vi "To and  From CSV.vi"() -> (0 "error out":errorcluster, 3 "Pass":bool)   [LabVIEW 2015, in "DAQmx Module Tests.lvlib"]
uses:
  DAQmx Module Tests.lvlib
  <vilib>/NI/Module Execution Interface/Engine Configuration/engine configuration.lvclass
  editor node/DAQmx Module editor node.lvclass
  <vilib>/NI/Configuration Framework/serializable configuration/NISE_CEF_serializable configuration.lvclass/NISE_CEF_serializable configuration.ctl
  module/configuration/Daqmx Module configuration.lvclass/Daqmx Module configuration.ctl
  <vilib>/Utility/LVClass/Get LV Class Name.vi
  <vilib>/NI/Configuration Framework/error generator/NISE_error generator.vi
  <vilib>/NI/Tag Bus Module Framework/channel/TBM channel.lvclass
  module/configuration/Daqmx Module configuration.lvclass
  <vilib>/NI/Configuration Framework/serializable configuration/NISE_CEF_serializable configuration.lvclass
panel:
  out "Object":bool
  out "Lines":bool
  out "Write Channels":bool
  out "Read Channels":bool
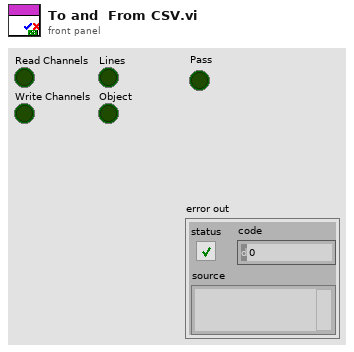
[diagram p1: front panel]
types:
  T1 = typedef "DAQmx Module Configuration.lvclass/Line.ctl" = cluster{"Channel Array":refnum<class "TBM channel.lvclass">[], "Physical Channel":string, "Measurement Type":T2, "Parameters":T3}
  T2 = typedef "DAQmx Module Configuration.lvclass/Measurement Type.ctl" = enum16{"Digital Input", "Digital Output", "Voltage Input", "Voltage Output", "Current Input", "Current Output", "RTD", "Thermocouple", "Strain", "PWM"}
  T3 = typedef "DAQmx Module Configuration.lvclass/Parameters.ctl" = cluster{"Digital Config":cluster{"Invert Lines?":bool}, "Voltage Config":cluster{"Maximum Value (V)":dbl, "Minimum Value (V)":dbl, "in terminal configuration (V)":i32, "out terminal configuration (V)":i32}, "Current Config":cluster{"Maximum Value (A)":dbl, "Minimum Value (A)":dbl, "shunt resistor location":i32, "input terminal configuration (C)":i32, "external shunt resistor value":dbl}, "RTD Config":cluster{"Maximum Value (°C)":dbl, "Minimum Value (°C)":dbl, "resistance configuration":i32, "r0":dbl, "current excitation value":dbl, "rtd type":i32, "current excitation source":i32}, "Thermocouple Config":cluster{"Minimum Value (C)":dbl, "Maximum Value (C)":dbl, "thermocouple type":i32, "cjc source":i32, "cjc value":dbl}, "Strain Config":cluster{"Maximum Value":dbl, "Minimum Value":dbl, "bridge information":cluster{"strain configuration":i32, "lead wire resistance":dbl, "initial bridge voltage":dbl, "voltage excitation source":i32, "voltage excitation value":dbl}, "strain gage information":cluster{"gage factor":dbl, "nominal gage resistance":dbl, "poisson ratio":dbl}}, "PWM Config":cluster{"Idle State":bool}}
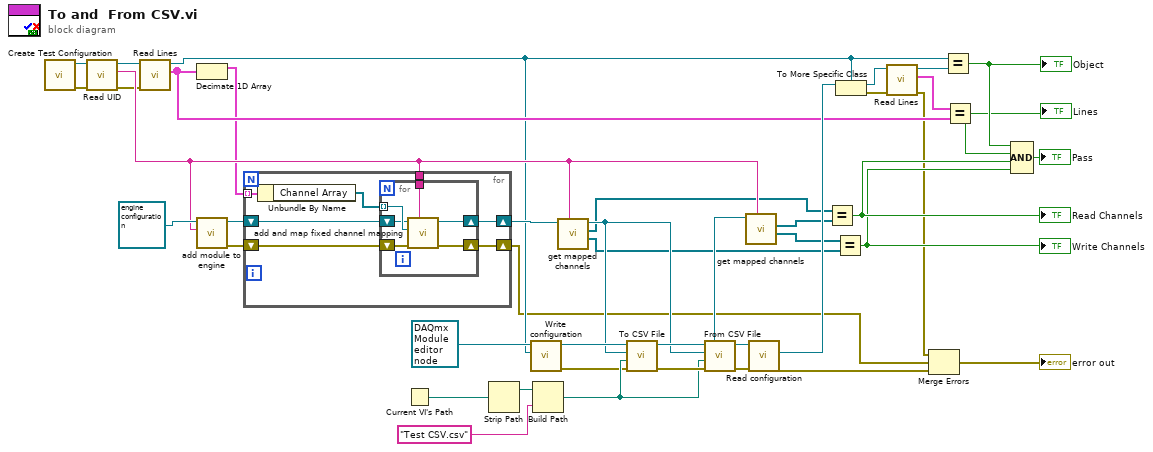
[diagram p0: block diagram]
diagram:
  n1 = call "Create Test Configuration.vi"() -> ("error out"=w17:errorcluster, "Module Configuration"=w27:refnum<class "Daqmx Module configuration.lvclass">)  [unwired: 7 in, 3 out]
  n2 = call <vilib>:"Read UID.vi"("error in"=w17, "configuration in"=w27) -> ("error out"=w13:errorcluster, "instance id"=w23:string, "configuration out"=w16:refnum<class "Daqmx Module configuration.lvclass">)  [unwired: 7 in]
  n3 = call "Read Lines.vi"("error in (no error)"=w13, "Daqmx Module configuration in"=w16) -> ("Lines"=w30:T1[], "Daqmx Module configuration out"=w15:refnum<class "Daqmx Module configuration.lvclass">)  [unwired: 7 in, 1 out]
  n4 = Decimate 1D Array(w30) -> (w18:T1[])  [unwired: 1 out]
  n5 = call-dynamic "add module to engine.vi"("module ID"=w23, "engine configuration in"=refnum<class "engine configuration.lvclass"> refnum ("engine configuration")) -> ("error out"=w12:errorcluster, "engine configuration out"=w28:refnum<class "engine configuration.lvclass">)  [unwired: 8 in]
  n6 = for {
    tunnel: w18 -> [w50] mode=indexing
    shift-right: [w48] -> w26
    shift-left: w28 -> [w47]
    tunnel: w23 -> [w46]
    shift-right: [w44] -> w9
    shift-left: w12 -> [w45]
    n7 = Unbundle By Name(w50) -> ("Channel Array"=w49:refnum<class "TBM channel.lvclass">[])
    n8 = for {
      tunnel: w49 -> [w56] mode=indexing
      tunnel: w46 -> [w53]
      shift-right: [w55] -> w48
      shift-left: w47 -> [w54]
      shift-right: [w51] -> w44
      shift-left: w45 -> [w52]
      n9 = call <vilib>:"add and map fixed channel mapping.vi"("module instance"=w53, "error in"=w52, "fixed channel"=w56, "engine configuration in"=w54) -> ("error out"=w51:errorcluster, "engine configuration out"=w55:refnum<class "engine configuration.lvclass">)  [unwired: 6 in]
    }
  }
  n10 = Current VI's Path() -> (path=w20:path)
  n11 = Strip Path(path=w20) -> (stripped path=w19:path)  [unwired: 1 out]
  n12 = call-dynamic "Write configuration.vi"("configuration"=w15, "Daqmx Module editor node in"=refnum<class "DAQmx Module editor node.lvclass"> refnum ("Daqmx Module editor node")) -> ("error out"=w5:errorcluster, "Daqmx Module editor node out"=w35:refnum<class "DAQmx Module editor node.lvclass">)  [unwired: 8 in]
  n13 = Build Path(base path=w19, name or relative path="Test CSV.csv") -> (appended path=w21:path)
  n14 = call-dynamic "get mapped channels.vi"("owner"=w23, "engine configuration in"=w26) -> ("write channels"=w4:refnum<class "TBM channel.lvclass">[], "read channels"=w3:refnum<class "TBM channel.lvclass">[], "engine configuration out"=w25:refnum<class "engine configuration.lvclass">)  [unwired: 5 in, 2 out]
  n15 = call-dynamic "To CSV File.vi"("error in (no error)"=w5, "Path"=w21, "engine configuration"=w25, "DAQmx Module Editor Node in"=w35) -> ("error out"=w38:errorcluster, "DAQmx Module Editor Node out"=w37:refnum<class "DAQmx Module editor node.lvclass">)  [unwired: 6 in]
  n16 = call-dynamic "From CSV File.vi"("error in (no error)"=w38, "Path"=w21, "engine configuration"=w25, "DAQmx Module Editor Node in"=w37) -> ("error out"=w34:errorcluster, "engine out"=w24:refnum<class "engine configuration.lvclass">, "DAQmx Module Editor Node out"=w33:refnum<class "DAQmx Module editor node.lvclass">)  [unwired: 4 in, 1 out]
  n17 = call-dynamic "get mapped channels.vi"("owner"=w23, "engine configuration in"=w24) -> ("write channels"=w1:refnum<class "TBM channel.lvclass">[], "read channels"=w2:refnum<class "TBM channel.lvclass">[])  [unwired: 5 in, 3 out]
  n18 = call-dynamic "Read configuration.vi"("error in"=w34, "Daqmx Module editor node in"=w33) -> ("error out"=w8:errorcluster, "configuration"=w32:refnum<class "NISE_CEF_serializable configuration.lvclass">)  [unwired: 7 in, 1 out]
  n19 = Equal?(x=w3, y=w2) -> (x = y?=w11:bool)
  "Read Channels" <- w11
  n20 = Equal?(x=w1, y=w4) -> (x = y?=w10:bool)
  "Write Channels" <- w10
  n21 = To More Specific Class(target class=w15, reference=w32) -> (specific class reference=w31:refnum<class "Daqmx Module configuration.lvclass">, error out=w14:errorcluster)  [unwired: 1 in]
  n22 = call "Read Lines.vi"("error in (no error)"=w14, "Daqmx Module configuration in"=w31) -> ("error out"=w7:errorcluster, "Lines"=w39:T1[], "Daqmx Module configuration out"=w43:refnum<class "Daqmx Module configuration.lvclass">)  [unwired: 7 in]
  n23 = Merge Errors(w7, w9, w8) -> (→"error out":errorcluster)
  n24 = Equal?(x=w15, y=w43) -> (x = y?=w42:bool)
  "Object" <- w42
  n25 = Equal?(x=w39, y=w30) -> (x = y?=w41:bool)
  "Lines" <- w41
  n26 = Compound Arithmetic op=AND(w42, w41, w11, w10) -> (→"Pass":bool)
